vi "RemoteVI Landing Page.vi"(0 "status":T1(array[cluster])) -> (4 "html":string)   [LabVIEW 2020, in "RemoteVI.lvlib"]
doc: "The landing page of RemoteVI Server (served on its own port with its own access token): every RUNNING share of status (RemoteVI Status.vi) as a link with its token, the target's name, kind, port and whether it is reachable from the whole network or view only; Nothing is shared right now. when none runs. Names and links are HTML-escaped (RemoteVI HTML Escape.vi). Pure function, cannot fail. Reference: landingPage() in tools\\lib\\server-app.mjs, vectors tests\\vectors\\server-app.json (landing)."
uses:
  RemoteVI.lvlib
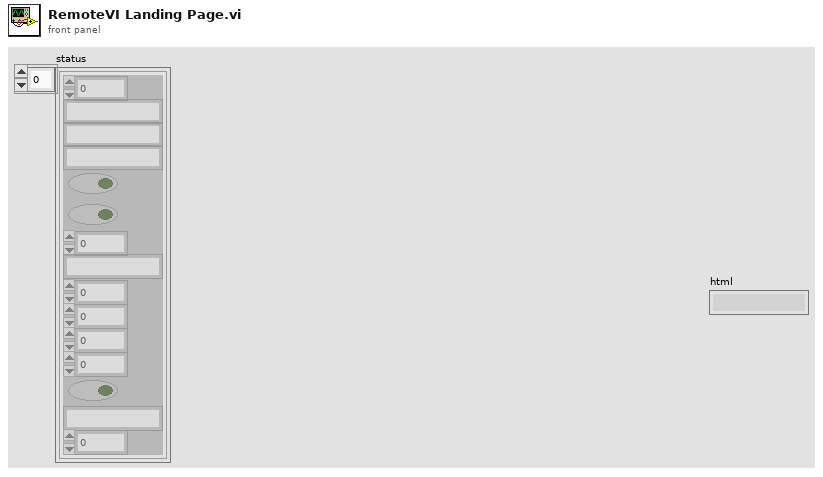
[diagram p1: front panel]
types:
  T1 = cluster{"port":u16, "url":string, "target":string, "kind":string, "whole network":bool, "running":bool, "uptime s":dbl, "clients":cluster{"address":string, "connected s":dbl, "idle s":dbl}[], "fps":dbl, "kB per s":dbl, "frames":u32, "latency ms":dbl, "view only":bool, "last error":string, "hWnd":u64}[]
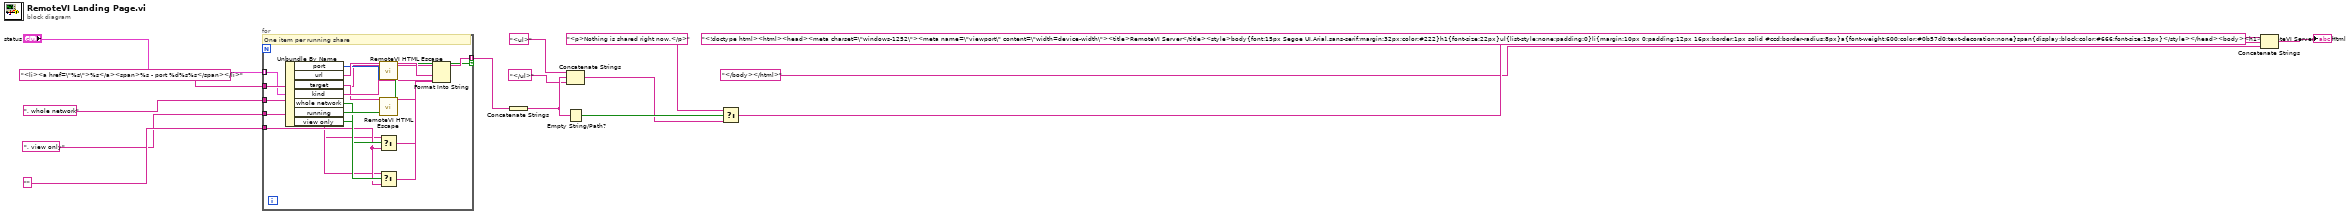
[diagram p0: block diagram]
diagram:
  n1 = for {
    tunnel: "status" -> [w17] mode=indexing
    tunnel: "<li><a href=\"%s\">%s</a><span>%s - port %d%s%s</span></li>" -> [w18]
    tunnel: ", whole network" -> [w19]
    tunnel: ", view only" -> [w20]
    tunnel: "" -> [w21]
    tunnel: [w33] -> w11 mode=indexing if=w27
    # "One item per running share"
    n2 = Unbundle By Name(w17) -> ("port"=w22:u16, "url"=w23:string, "target"=w24:string, "kind"=w25:string, "whole network"=w26:bool, "running"=w27:bool, "view only"=w28:bool)
    n3 = call "RemoteVI HTML Escape.vi"("text"=w23) -> ("html"=w29:string)  [unwired: 14 in]
    n4 = call "RemoteVI HTML Escape.vi"("text"=w24) -> ("html"=w30:string)  [unwired: 14 in]
    n5 = Select(t=w19, s=w26, f=w21) -> (s? t:f=w31:string)
    n6 = Select(t=w20, s=w28, f=w21) -> (s? t:f=w32:string)
    n7 = Format Into String(format string=w18, w29, w30, w25, w22, w31, w32) -> (resulting string=w33:string)  [unwired: 2 in, 1 out]
  }
  n8 = Concatenate Strings(w11) -> (w12:string)
  n9 = Concatenate Strings("<ul>", w12, "</ul>") -> (w13:string)
  n10 = Empty String/Path?(string/path=w12) -> (empty?=w14:bool)
  n11 = Select(t="<p>Nothing is shared right now.</p>", s=w14, f=w13) -> (s? t:f=w15:string)
  n12 = Concatenate Strings("<!doctype html><html><head><meta charset=\"windows-1252\"><meta name=\"viewport\" content=\"width=device-width\"><title>RemoteVI Server</title><style>body{font:15px Segoe UI,Arial,sans-serif;margin:32px;color:#222}h1{font-size:22px}ul{list-style:none;padding:0}li{margin:10px 0;padding:12px 16px;border:1px solid #ccd;border-radius:8px}a{font-weight:600;color:#0b57d0;text-decoration:none}span{display:block;color:#666;font-size:13px}</style></head><body><h1>RemoteVI Server</h1>", w15, "</body></html>") -> (→"html":string)
